vi "clone.vi"(0 "reference":refnum<class "ChoiceNode.lvclass">, 5 "error in (no error)":errorcluster) -> (14 "reference out":refnum<class "ChoiceNode.lvclass">, 15 "clonedInterfaceNode":refnum<class "AbstractNode.lvclass">, 19 "error out":errorcluster)   [LabVIEW 2020, in "ChoiceNode.lvclass"]
doc: "public Object clone()"
uses:
  <resource>/Framework/Providers/Open_GDS/UML/ChoiceNode_class/ChoiceNode.lvclass
  C:/Program Files (x86)/National Instruments/LabVIEW 2020/resource/Framework/Providers/Open_GDS/UML/RectangularNode_class/RectangularNode.lvclass
  C:/Program Files (x86)/National Instruments/LabVIEW 2020/resource/Framework/Providers/Open_GDS/UML/AbstractNode_class/AbstractNode.lvclass
  <resource>/Framework/Providers/Open_GDS/UML/AbstractNode_class/AbstractNode.lvclass
  <resource>/Framework/Providers/Open_GDS/UML/MultiLineString_class/MultiLineString.lvclass
  <resource>/Framework/Providers/Open_GDS/UML/RectangularNode_class/RectangularNode.lvclass
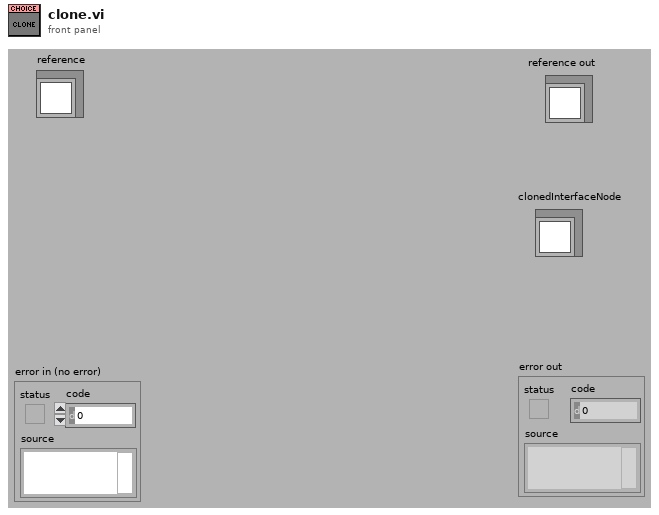
[diagram p1: front panel]
types:
  T1 = typedef "RectangularNode.lvclass/ObjectAttributes.ctl" = cluster{"bounds":T2}
  T2 = typedef "Rectangle Rectangle2D.ctl" = cluster{"x":dbl, "y":dbl, "width":dbl, "height":dbl}
  T3 = typedef "ChoiceNode.lvclass/ObjectAttributes.ctl" = cluster{"Text":refnum<class "MultiLineString.lvclass">, "DEFAULT_WIDTH":i32, "DEFAULT_HEIGHT":i32}
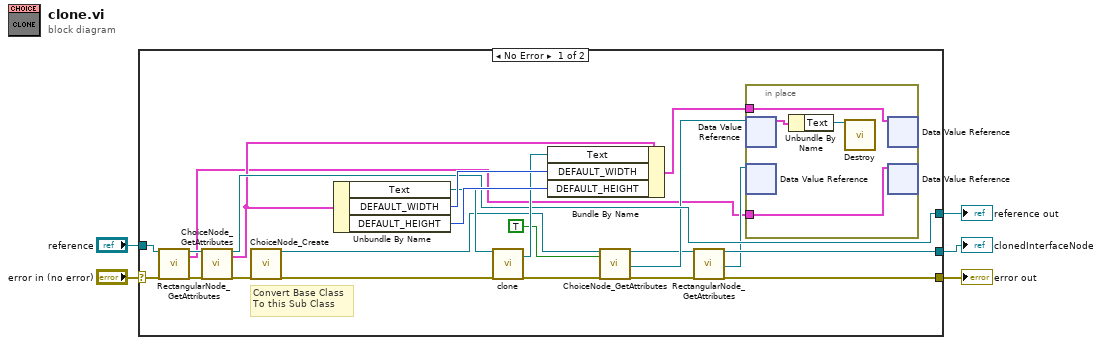
[diagram p0: block diagram]
diagram:
  n1 = case shown="No Error" "error in (no error)" {
    selector: "error in (no error)" -> [w28 w33]
    tunnel: "reference" -> [w12 w34]
    tunnel: [w10 w33] -> w4
    tunnel: [w20 w34] -> w3
    tunnel: [w8 _] -> w1
    frame No Error {
      # "Convert Base Class\nTo this Sub Class"
      n2 = call <resource>:"RectangularNode_GetAttributes.vi"("reference in"=w12, "error in (no error)"=w28) -> ("reference out"=w11:refnum<class "ChoiceNode.lvclass">, "Data"=w6:T1, "error out"=w13:errorcluster)  [unwired: 14 in, 1 out]
      n3 = call <resource>:"ChoiceNode_GetAttributes.vi"("reference in"=w11, "error in (no error)"=w13) -> ("reference out"=w20:refnum<class "ChoiceNode.lvclass">, "Data"=w17:T3, "error out"=w19:errorcluster)  [unwired: 1 in, 14 out]
      n4 = call <resource>:"ChoiceNode_Create.vi"("error in (no error)"=w19) -> ("reference out"=w21:refnum<class "ChoiceNode.lvclass">, "error out"=w25:errorcluster)  [unwired: 17 in]
      n5 = Unbundle By Name(w17) -> ("Text"=w24:refnum<class "MultiLineString.lvclass">, "DEFAULT_WIDTH"=w27:i32, "DEFAULT_HEIGHT"=w26:i32)
      n6 = call-dynamic "clone.vi"("reference"=w24, "error in (no error)"=w25) -> ("clonedMultiLineString"=w23:refnum<class "MultiLineString.lvclass">, "error out"=w22:errorcluster)  [unwired: 15 in, 1 out]
      n7 = Bundle By Name(cluster=w17, "Text"=w23, "DEFAULT_WIDTH"=w27, "DEFAULT_HEIGHT"=w26) -> (w14:T3)
      n8 = call <resource>:"ChoiceNode_GetAttributes.vi"("reference in"=w21, "OnlyGetDvrReference(False)"=TRUE, "error in (no error)"=w22) -> ("reference out"=w9:refnum<class "ChoiceNode.lvclass">, "DataRef"=w15:refnum<data-value>, "error out"=w16:errorcluster)  [unwired: 13 in, 1 out]
      n9 = call <resource>:"RectangularNode_GetAttributes.vi"("reference in"=w9, "error in (no error)"=w16) -> ("reference out"=w8:refnum<class "ChoiceNode.lvclass">, "DataRef"=w7:refnum<data-value>, "error out"=w10:errorcluster)  [unwired: 14 in, 1 out]
      n10 = in-place {
        in-place-border: w14 -> [w32]
        in-place-border: w6 -> [w29]
        n11 = in-place-dvr #1(w15) -> (w30:T3)  [unwired: 1 out]
        n12 = in-place-dvr #2(w7) -> ()  [unwired: 2 out]
        n13 = Unbundle By Name(w30) -> ("Text"=w31:refnum<class "MultiLineString.lvclass">)
        n14 = call-dynamic "Destroy.vi"("reference"=w31) -> ()  [unwired: 17 in, 2 out]
        n15 = in-place-dvr #1(w32) -> ()  [unwired: 2 out]
        n16 = in-place-dvr #2(w29) -> ()  [unwired: 2 out]
      }
    }
    frame Error {
    }
  }
  "reference out" <- w3
  "error out" <- w4
  "clonedInterfaceNode" <- w1
